vi "case selector.vi"() -> ()   [LabVIEW 2018]
panel:
  in  "Condition":bool
  out "x-y":dbl
  in  "x 2":dbl
  in  "y 2":dbl
  out "x+y":dbl
  in  "x":dbl
  in  "y":dbl
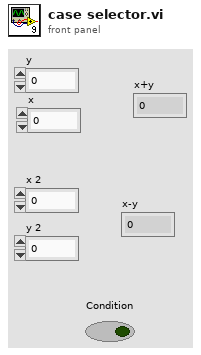
[diagram p1: front panel]
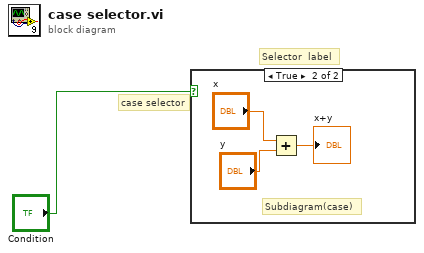
[diagram p0: block diagram]
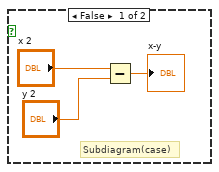
[diagram p2: hidden frame]
diagram:
  # "case selector"
  # "Selector  label"
  n1 = case shown="True" "Condition" {
    frame False {
      # "Subdiagram(case)"
      n2 = Subtract(x="x 2", y="y 2") -> (x-y=→"x-y":dbl)
    }
    frame True {
      # "Subdiagram(case)"
      n3 = Add(x="x", y="y") -> (x+y=→"x+y":dbl)
    }
  }
